vi "execute HO.vi"(8 "error in (no error)":errorcluster caption="에러 입력(에러 없음)", 11 "NR 입력":refnum<class "NR.lvclass">) -> (0 "error out":errorcluster caption="에러 출력", 3 "NR 출력":refnum<class "NR.lvclass">)   [LabVIEW 2023, in "ANRITSU Call Box.lvlib" / "NR.lvclass"]
uses:
  NR.lvclass
  NR.lvclass/NR.ctl
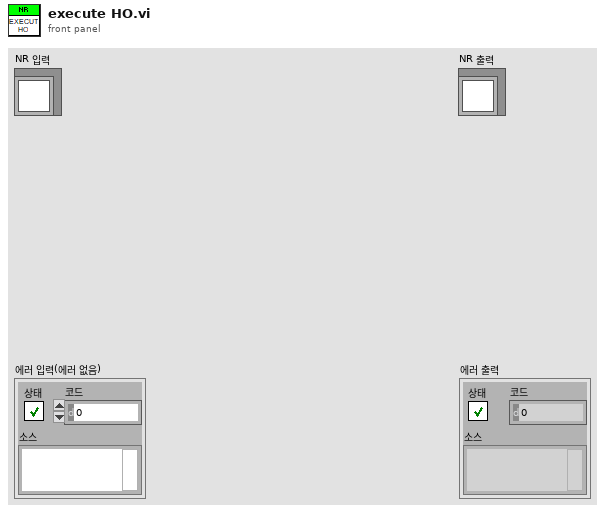
[diagram p1: front panel]
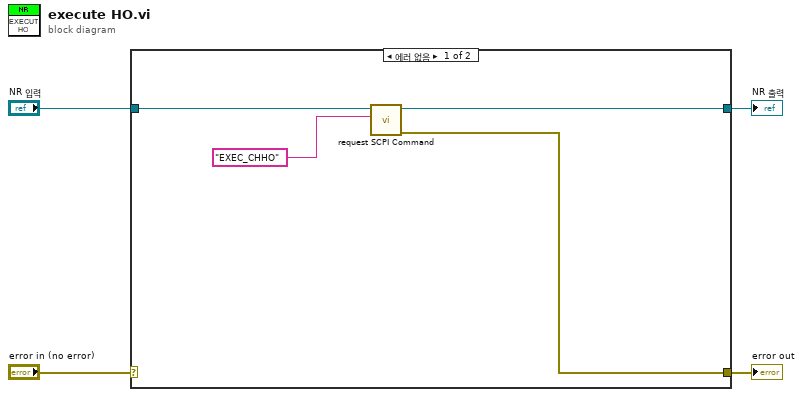
[diagram p0: block diagram]
diagram:
  n1 = case shown="에러 없음" "error in (no error)" {
    selector: "error in (no error)" -> [_ w10]
    tunnel: [w5 w10] -> w3
    tunnel: [w6 w9] -> w1
    tunnel: "NR 입력" -> [w8 w9]
    frame No Error {
      n2 = call "request SCPI Command.vi"("SCPI Command"="EXEC_CHHO", "NR in"=w8) -> ("error out"=w5:errorcluster, "NR out"=w6:refnum<class "NR.lvclass">)  [unwired: 8 in]
    }
    frame Error {
    }
  }
  "error out" <- w3
  "NR 출력" <- w1
